vi "File Buffer.vi"(10 "File Buffer In":cluster{"Path":path, "Data Series":T1[]}, 11 "Operation":enum16{"Get", "Set"}(ring)) -> (2 "File Buffer Out":cluster{"Path":path, "Data Series":T1[]})   [LabVIEW 2020, in "Data Viewer.lvlib" / "Data Viewer.lvclass"]
uses:
  Data Viewer.lvclass
  Data Serie--cluster.ctl
  Data Viewer.lvlib
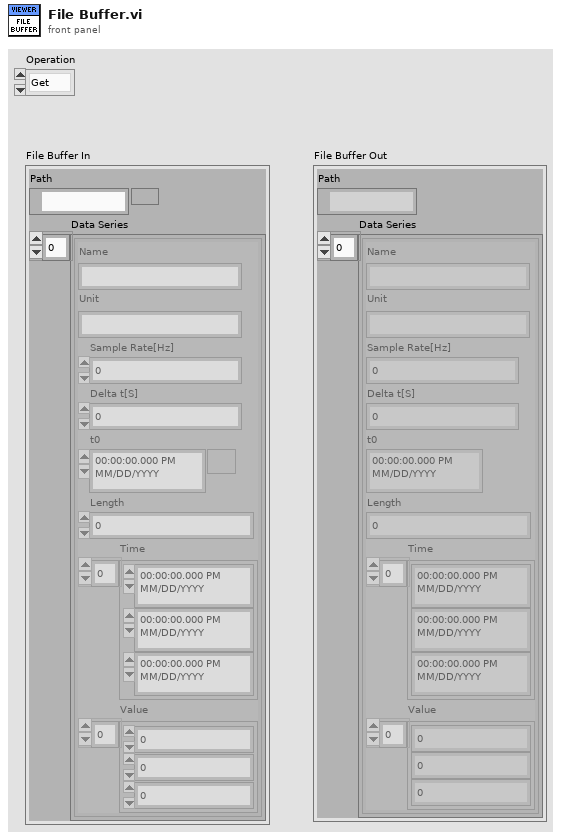
[diagram p1: front panel]
types:
  T1 = typedef "Data Viewer.lvlib/Data Serie--cluster.ctl" = cluster{"Name":string, "Unit":string, "Sample Rate[Hz]":dbl, "Delta t[S]":dbl, "t0":timestamp, "Length":i32, "Time":timestamp[], "Value":dbl[]}
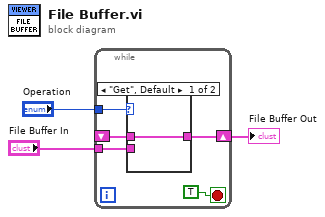
[diagram p0: block diagram]
diagram:
  n1 = while {
    tunnel: "File Buffer In" -> [w7]
    tunnel: "Operation" -> [w6]
    shift-right: [w5] -> w1
    shift-left: _ -> [w4]
    stop <- TRUE stop-if-true
    n2 = case shown="\"Get\", Default" w6 {
      tunnel: w7 -> [_ w10]
      tunnel: [w9 w10] -> w5
      tunnel: w4 -> [w9 _]
      frame "Get", Default {
      }
      frame "Set" {
      }
    }
  }
  "File Buffer Out" <- w1
